vi "VIH - VI Doc Editor #2 - Build Control Tree.vi"(6 "Ctrl Attributes":T1[](array[typedef]), 7 "Expand Tab Control (F)":bool, 8 "error in":errorcluster, 9 "Parent tag":string, 10 "Tree Refnum":refnum<vi>, 11 "Ctrl Refnums":refnum<vi>[](array[refnum])) -> (0 "error out":errorcluster, 2 "Controls Info":T2[](array[typedef]), 3 "dup Ctrl Refnums":refnum<vi>[](array[refnum]))   [LabVIEW 2014]
doc: "::: VI Helpeks :::\nCopyright (c) 2000-2026 Konstantin Shifershteyn. All rights reserved."
uses:
  VIH - VI Doc Editor #2 Typedef - Info Cluster.ctl
  _VIH HelpGen.llb/VIH HelpGen Typedef - Control Terminal Attributes Cluster.ctl
panel:
  # "VI Helpeks\nCopyright (c) 2012-2026 Konstantin Shifershteyn"
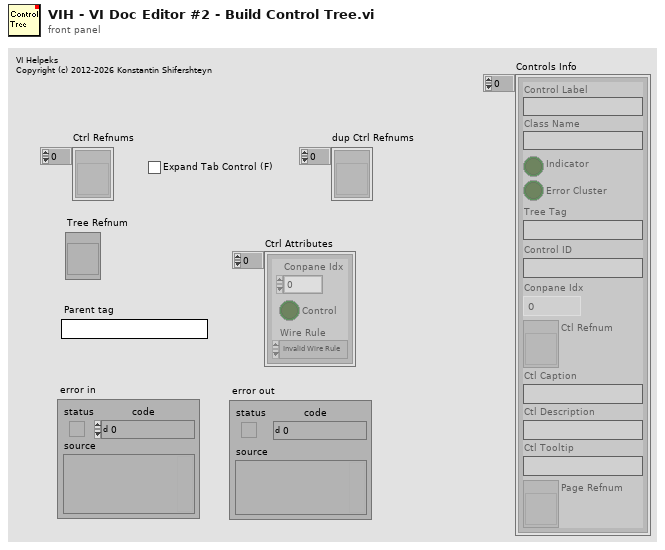
[diagram p1: front panel]
types:
  T1 = typedef "VIH HelpGen Typedef - Control Terminal Attributes Cluster.ctl" = cluster{"Conpane Idx":i32, "Control":bool, "Wire Rule":enum16{"Invalid Wire Rule", "Required", "Recommended", "Optional", "Dynamic Dispatch"}}
  T2 = typedef "VIH - VI Doc Editor #2 Typedef - Info Cluster.ctl" = cluster{"Control Label":string, "Class Name":string, "Indicator":bool, "Error Cluster":bool, "Tree Tag":string, "Control ID":string, "Conpane Idx":i32, "Ctl Refnum":refnum<vi>, "Ctl Caption":string, "Ctl Description":string, "Ctl Tooltip":string, "Page Refnum":refnum<vi>}
  T3 = cluster{"Left Cell":string, "Child Text":string[], "Child tag":string, "Symbol":i32}
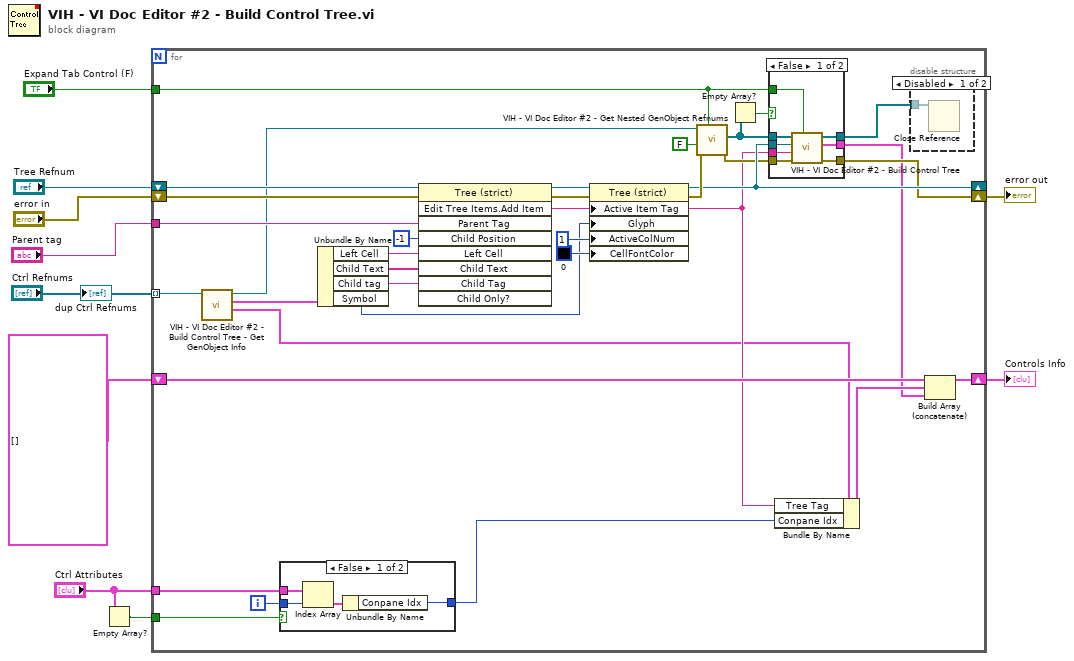
[diagram p0: block diagram]
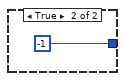
[diagram p3: hidden frame]
diagram:
  n1 = Empty Array?(array="Ctrl Attributes") -> (empty?=w5:bool)
  n2 = for {
    tunnel: "Ctrl Refnums" -> [w18] mode=indexing
    shift-right: [w35] -> _
    shift-left: "Tree Refnum" -> [w41]
    shift-right: [w31] -> w4
    shift-left: "error in" -> [w39]
    tunnel: "Parent tag" -> [w38]
    shift-right: [w29] -> w1
    shift-left: T2[] [] ("Controls Info") -> [w30]
    tunnel: "Ctrl Attributes" -> [w25]
    tunnel: w5 -> [w23]
    tunnel: "Expand Tab Control (F)" -> [w20]
    i -> [w24]
    n3 = call "VIH - VI Doc Editor #2 - Build Control Tree - Get GenObject Info.vi"("Gen Refnum"=w18) -> ("Info"=w11:T2, "Tree data"=w16:T3, "dup Gen Refnum"=w17:refnum<vi>)  [unwired: 8 in]
    n4 = case shown="False" w23 {
      tunnel: w25 -> [w49 _]
      tunnel: w24 -> [w48 _]
      tunnel: [w46 -1 ("Conpane Idx")] -> w22
      frame False {
        n5 = Index Array(array=w49, index=w48) -> (element=w47:T1)
        n6 = Unbundle By Name(w47) -> ("Conpane Idx"=w46:i32)
      }
      frame True {
      }
    }
    n7 = Unbundle By Name(w16) -> ("Left Cell"=w15:string, "Child Text"=w14:string[], "Child tag"=w13:string, "Symbol"=w12:i32)
    n8 = invoke on="Invoke Node" class="Tree (strict)" method="Edit Tree Items.Add Item"(reference=w41, error in=w39, "Parent Tag"=w38, "Child Position"=-1, "Left Cell"=w15, "Child Text"=w14, "Child Tag"=w13) -> (reference out=w42:refnum<vi>, error out=w43:errorcluster, "Edit Tree Items:Add Item"=w26:string)  [unwired: 2 in, 6 out]
    n9 = property on="Property Node" class="Tree (strict)"(reference=w42, error in=w43, "Active Item Tag"=w26, "Glyph"=w12, "ActiveColNum"=1 ("Active Cell:Active Column Number"), "CellFontColor"=u32 0) -> (reference out=w35:refnum<vi>, error out=w37:errorcluster)
    n10 = call "VIH - VI Doc Editor #2 - Get Nested GenObject Refnums.vi"("Expand Tab Control (T)"=w20, "error in"=w37, "Skip Cluster if it's Array element (F)"=FALSE ("Skip Cluster if it's Array element (T)"), "Gen Refnum"=w17) -> ("error out"=w34:errorcluster, "Gen Refnums"=w36:refnum<vi>[])  [unwired: 5 in, 1 out]
    n11 = Empty Array?(array=w36) -> (empty?=w33:bool)
    n12 = case shown="False" w33 {
      tunnel: w36 -> [w58 w60]
      tunnel: w35 -> [w57 _]
      tunnel: w26 -> [w56 _]
      tunnel: w34 -> [w55 w59]
      tunnel: [w54 w60] -> w32
      tunnel: [w53 w59] -> w31
      tunnel: [w52 _] -> w27
      tunnel: w20 -> [w51 _]
      frame False {
        n13 = call "VIH - VI Doc Editor #2 - Build Control Tree.vi"("Expand Tab Control (F)"=w51, "error in"=w55, "Parent tag"=w56, "Tree Refnum"=w57, "Ctrl Refnums"=w58) -> ("error out"=w53:errorcluster, "Controls Info"=w52:T2[], "dup Ctrl Refnums"=w54:refnum<vi>[])  [unwired: 4 in]
      }
      frame True {
      }
    }
    n14 = Bundle By Name(cluster=w11, "Tree Tag"=w26, "Conpane Idx"=w22) -> (w28:T2)
    n15 = disable-structure shown="Disabled" {
      disable-tunnel: w32 -> [w45 _]
      frame Disabled {
        n16 = Close Reference(reference=w45) -> ()  [unwired: 1 in, 1 out]
      }
      frame Enabled {
      }
    }
    n17 = Build Array (concatenate)(w30, w28, w27) -> (w29:T2[])
  }
  "error out" <- w4
  "Controls Info" <- w1
  "dup Ctrl Refnums" <- "Ctrl Refnums"
